vi "VideoWriter_Probe.vi"(11 "OpenLvVision_OpenCv.lvlib:VideoWriter":refnum<class "VideoWriter.lvclass">) -> (2 "Value String":string, 3 "Pause VI":bool)   [LabVIEW 2020, in "OpenLvVision_OpenCv.lvlib" / "VideoWriter.lvclass"]
uses:
  _LvHelpers/EdvrObject/EdvrObject.lvclass/EdvrObject.ctl
  VideoWriter.lvclass
  _LvHelpers/EdvrObject/EdvrObject.lvclass
  C:/Users/lukas/Downloads/OpenLvVision_OpenCv/SourceCode/LabView/OpenLvVision_OpenCv/_LvHelpers/EdvrObject/EdvrObject.lvclass
  C:/Users/lukas/Downloads/OpenLvVision_OpenCv/SourceCode/LabView/OpenLvVision_OpenCv/VideoIO/VideoWriter/VideoWriter.lvclass
panel:
  out "BackendName":string
  out "Open":bool
  out "Reference":u64 format="%.0x"
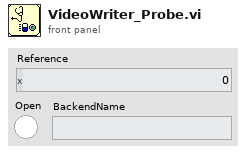
[diagram p1: front panel]
types:
  T1 = typedef "OpenLvVision_OpenCv.lvlib/EdvrObject.lvclass/Edvr.ctl" = refnum<data-value>
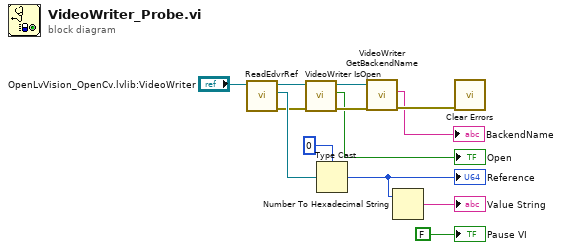
[diagram p0: block diagram]
diagram:
  n1 = call "ReadEdvrRef.vi"("EdvrObject in"="OpenLvVision_OpenCv.lvlib:VideoWriter") -> ("error out"=w3:errorcluster, "Edvr"=w9:T1, "EdvrObject out"=w4:refnum<class "VideoWriter.lvclass">)  [unwired: 8 in]
  n2 = call "VideoWriter IsOpen.vi"("error in (no error)"=w3, "VideoWriter in"=w4) -> ("error out"=w6:errorcluster, "Open"=→"Open":bool, "VideoWriter out"=w7:refnum<class "VideoWriter.lvclass">)  [unwired: 7 in]
  n3 = Type Cast(type=u64 0, x=w9) -> (*(type *) &x=w11:u64)
  "Reference" <- w11
  n4 = call "VideoWriter GetBackendName.vi"("error in (no error)"=w6, "VideoWriter in"=w7) -> ("error out"=w5:errorcluster, "BackendName"=→"BackendName":string)  [unwired: 7 in, 1 out]
  n5 = Number To Hexadecimal String(2:w11) -> (0:→"Value String":string)  [unwired: 1 in]
  n6 = call <vilib>:"Clear Errors.vi"("error in (no error)"=w5) -> ()  [unwired: 5 in, 2 out]
  "Pause VI" <- FALSE
